vi "Parse Connect FSV.vi"(7 "error in (no error)":errorcluster caption="에러 입력(에러 없음)", 9 "문자열":string, 10 "Instrument Manager 입력":refnum<class "Instrument Manager.lvclass">) -> (0 "error out":errorcluster caption="에러 출력", 1 "VISA Resource":refnum<visa-resource-name>, 2 "Connect FSV Param":T1, 3 "Instrument Manager 출력":refnum<class "Instrument Manager.lvclass">)   [LabVIEW 2023, in "Instrument Manager.lvclass"]
uses:
  Instrument Manager.lvclass
  Connect FSV Params.ctl
  Instrument Manager.lvclass/Instrument Manager.ctl
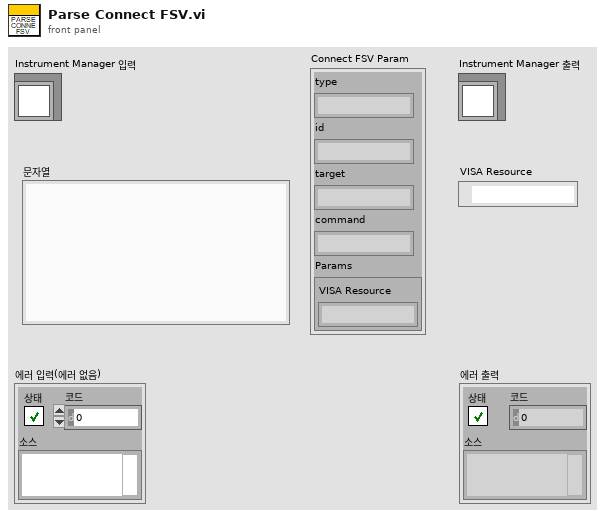
[diagram p1: front panel]
types:
  T1 = typedef "Instrument Manager.lvclass/Connect FSV Params.ctl" = cluster{"type":string, "id":string, "target":string, "command":string, "Params":cluster{"VISA Resource":string}}
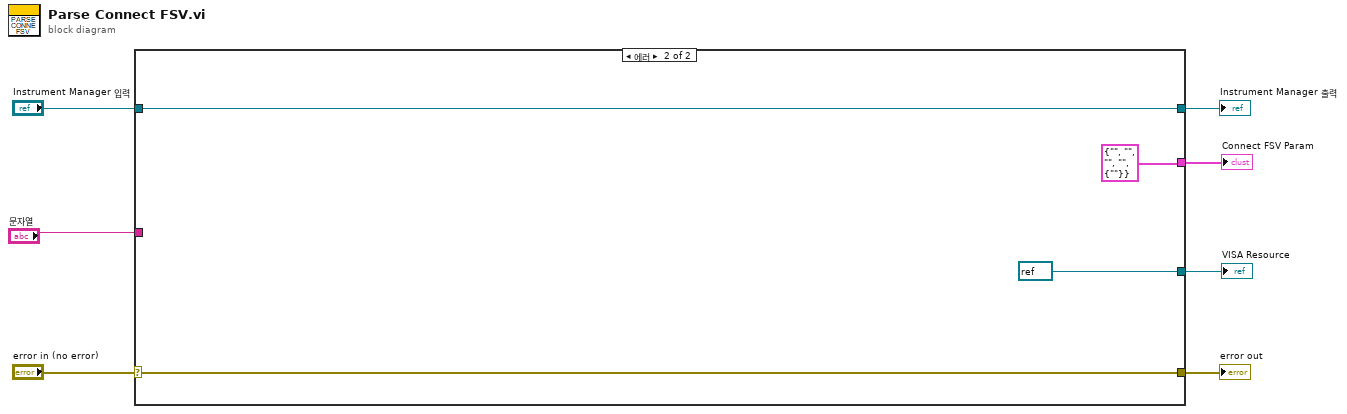
[diagram p0: block diagram]
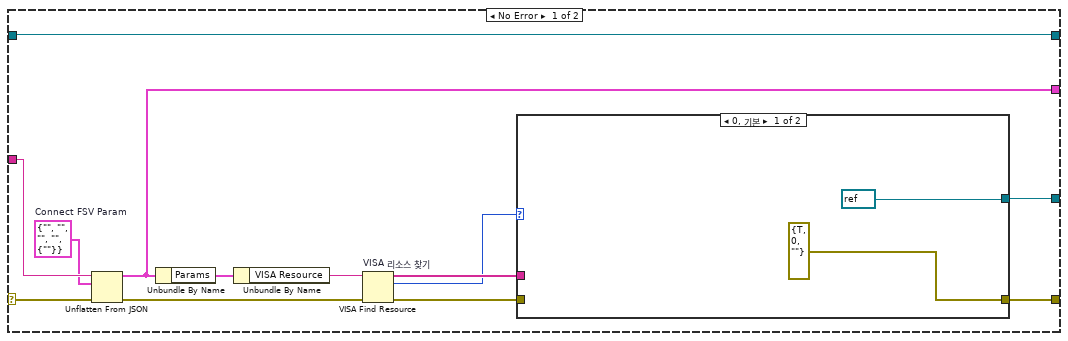
[diagram p2: hidden frame]
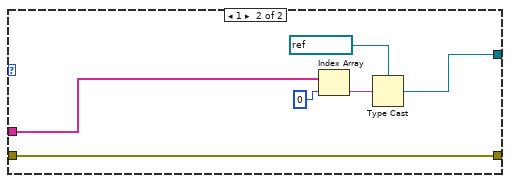
[diagram p3: hidden frame]
diagram:
  n1 = case shown="에러" "error in (no error)" {
    selector: "error in (no error)" -> [w17 w32]
    tunnel: [w9 w32] -> w6
    tunnel: [w20 w31] -> w4
    tunnel: "Instrument Manager 입력" -> [w20 w31]
    tunnel: "문자열" -> [w16 _]
    tunnel: [w12 refnum<visa-resource-name> refnum ("VISA 리소스 이름")] -> w2
    tunnel: [w8 T1 {"type"="", "id"="", "target"="", "command"="", "Params"={"VISA Resource"=""}} ("Connect FSV Param")] -> w1
    frame No Error {
      w15 = T1 {"type"="", "id"="", "target"="", "command"="", "Params"={"VISA Resource"=""}}  # Connect FSV Param
      n2 = Unflatten From JSON(JSON string=w16, type and defaults=w15, error in (no error)=w17) -> (value=w8:T1, error out=w14:errorcluster)  [unwired: 4 in]
      n3 = Unbundle By Name(w8) -> ("Params"=w19:cluster{"VISA Resource":string})
      n4 = Unbundle By Name(w19) -> ("VISA Resource"=w18:string)
      n5 = VISA Find Resource "VISA 리소스 찾기"(8:w14, 11:w18) -> (0:w10:errorcluster, 2:w11:u32, 3:w13:string[])  [unwired: 1 in]
      n6 = case shown="0, 기본" w11 {
        tunnel: w13 -> [_ w27]
        tunnel: [refnum<visa-resource-name> refnum ("VISA 리소스 이름") w24] -> w12
        tunnel: w10 -> [_ w23]
        tunnel: [errorcluster {"status"=TRUE, "code"=0, "source"=""} ("error out") w23] -> w9
        frame 0, Default {
        }
        frame 1 {
          n7 = Index Array(array=w27, index=0 ("인덱스")) -> (element=w26:string)
          n8 = Type Cast(type=refnum<visa-resource-name> "COM3" ("VISA 리소스 이름"), x=w26) -> (*(type *) &x=w24:refnum<visa-resource-name>)
        }
      }
    }
    frame Error {
    }
  }
  "error out" <- w6
  "Instrument Manager 출력" <- w4
  "VISA Resource" <- w2
  "Connect FSV Param" <- w1
